vi "UNITTESTS.vi"   [LabVIEW 2019]
uses:
  <vilib>/addons/_JKI Toolkits/Caraya/classes/Test/Test.lvclass
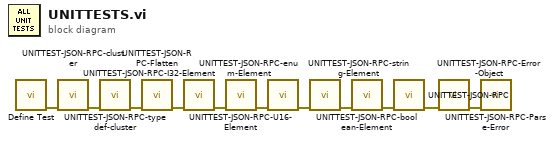
[diagram p0: block diagram]
diagram:
  n1 = call <vilib>:"Define Test.vi"() -> ("error out"=w11:errorcluster)  [unwired: 10 in, 1 out]
  n2 = call "UNITTEST-JSON-RPC-cluster.vi"("error in (no error)"=w11) -> ("error out"=w10:errorcluster)  [unwired: 10 in]
  n3 = call "UNITTEST-JSON-RPC-typedef-cluster.vi"("error in (no error)"=w10) -> ("error out"=w9:errorcluster)  [unwired: 10 in]
  n4 = call "UNITTEST-JSON-RPC-Flatten.vi"("error in (no error)"=w9) -> ("error out"=w4:errorcluster)  [unwired: 10 in]
  n5 = call "UNITTEST-JSON-RPC-I32-Element.vi"("error in (no error)"=w4) -> ("error out"=w8:errorcluster)  [unwired: 10 in]
  n6 = call "UNITTEST-JSON-RPC-U16-Element.vi"("error in (no error)"=w8) -> ("error out"=w7:errorcluster)  [unwired: 10 in]
  n7 = call "UNITTEST-JSON-RPC-enum-Element.vi"("error in (no error)"=w7) -> ("error out"=w6:errorcluster)  [unwired: 10 in]
  n8 = call "UNITTEST-JSON-RPC-string-Element.vi"("error in (no error)"=w6) -> ("error out"=w5:errorcluster)  [unwired: 10 in]
  n9 = call "UNITTEST-JSON-RPC-boolean-Element.vi"("error in (no error)"=w5) -> ("error out"=w3:errorcluster)  [unwired: 10 in]
  n10 = call "UNITTEST-JSON-RPC.vi"("error in (no error)"=w3) -> ("error out"=w2:errorcluster)  [unwired: 10 in]
  n11 = call "UNITTEST-JSON-RPC-Error-Object.vi"("error in (no error)"=w2) -> ("error out"=w1:errorcluster)  [unwired: 10 in]
  n12 = call "UNITTEST-JSON-RPC-Parse-Error.vi"("error in (no error)"=w1) -> ()  [unwired: 10 in, 1 out]
